vi "RDV-addDataToMap.vi"(7 "Use ignore list (false)":bool, 8 "error in (no error)":errorcluster, 9 "data":T2[](array[typedef]), 10 "all data":cluster{"key":string, "data":T1}[](array[cluster]), 11 "RDV-Reflection_Data_viewer in":refnum<class "RDV-Reflection_Data_viewer.lvclass">) -> (0 "error out":errorcluster, 3 "RDV-Reflection_Data_viewer out":refnum<class "RDV-Reflection_Data_viewer.lvclass">)   [LabVIEW 2020, in "RDV-Reflection_Data_viewer.lvclass"]
doc: "Adds data clusters with their keys to the viewer's data map. Use ignore list skips keys on the ignore list."
uses:
  RDV-Reflection_Data_viewer.lvclass
  Reflector/RFH-common_data_format.ctl
  RDV-DATA_MAP_CLUST.ctl
  RDV-Reflection_Data_viewer.lvclass/RDV-Reflection_Data_viewer.ctl
  Reflector/RFH-Reflection_File_Handler.lvlib
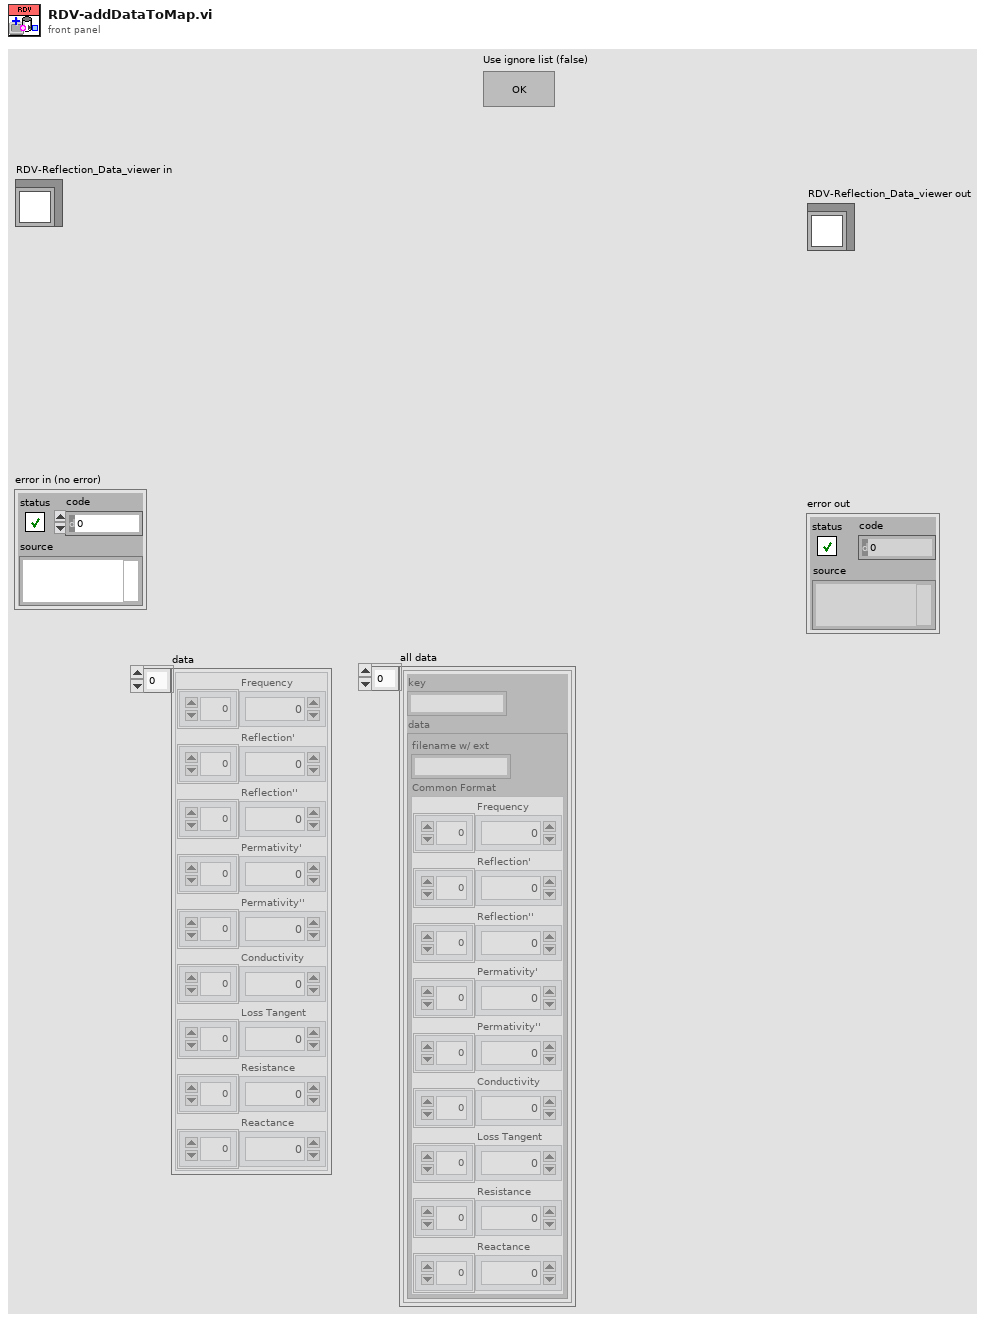
[diagram p1: front panel]
types:
  T1 = typedef "RDV-Reflection_Data_viewer.lvclass/RDV-DATA_MAP_CLUST.ctl" = cluster{"filename w/ ext":string, "Common Format":T2}
  T2 = typedef "RFH-Reflection_File_Handler.lvlib/RFH-common_data_format.ctl" = cluster{"Frequency":dbl[], "Reflection'":dbl[], "Reflection''":dbl[], "Permativity'":dbl[], "Permativity''":dbl[], "Conductivity":dbl[], "Loss Tangent":dbl[], "Resistance":dbl[], "Reactance":dbl[]}
  T3 = typedef "RDV-Reflection_Data_viewer.lvclass/RDV-UPDATE_IGNORE_LIST.ctl" = string[]
  T4 = typedef "RDV-Reflection_Data_viewer.lvclass/RDV-DATA_MAP.ctl" = map{string, T1}
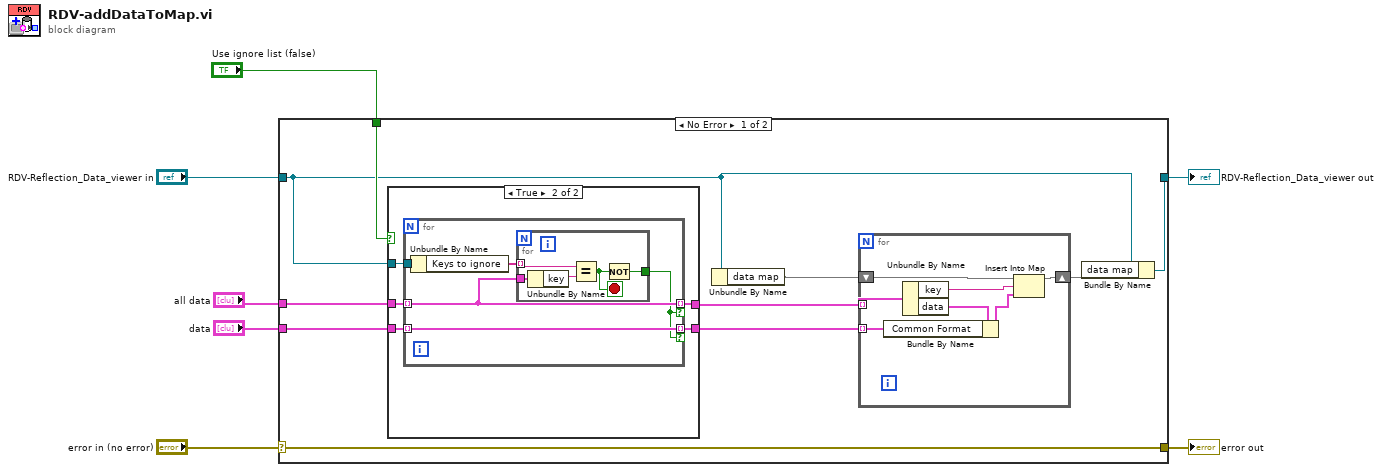
[diagram p0: block diagram]
diagram:
  n1 = case shown="No Error" "error in (no error)" {
    selector: "error in (no error)" -> [w14 w43]
    tunnel: [w14 w43] -> w6
    tunnel: [w15 w42] -> w4
    tunnel: "RDV-Reflection_Data_viewer in" -> [w8 w42]
    tunnel: "all data" -> [w12 _]
    tunnel: "data" -> [w13 _]
    tunnel: "Use ignore list (false)" -> [w9 _]
    frame No Error {
      n2 = case shown="True" w9 {
        tunnel: w13 -> [w18 w24]
        tunnel: w12 -> [w19 w23]
        tunnel: [w19 w22] -> w11
        tunnel: [w18 w21] -> w10
        tunnel: w8 -> [_ w20]
        frame False {
        }
        frame True {
          n3 = for {
            tunnel: w24 -> [w29] mode=indexing
            tunnel: w23 -> [w26] mode=indexing
            tunnel: [w26] -> w22 mode=indexing if=w25
            tunnel: [w29] -> w21 mode=indexing if=w25
            tunnel: w20 -> [w28]
            n4 = Unbundle By Name(w28) -> ("Keys to ignore"=w27:T3)
            n5 = for {
              tunnel: w27 -> [w32] mode=indexing
              tunnel: w26 -> [w34]
              tunnel: [w31] -> w25
              stop <- w30 stop-if-true
              n6 = Unbundle By Name(w34) -> ("key"=w33:string)
              n7 = Equal?(x=w32, y=w33) -> (x = y?=w30:bool)
              n8 = Not(x=w30) -> (.not. x?=w31:bool)
            }
          }
        }
      }
      n9 = Unbundle By Name(w8) -> ("data map"=w17:T4)
      n10 = for {
        shift-right: [w40] -> w16
        shift-left: w17 -> [w41]
        tunnel: w11 -> [w39] mode=indexing
        tunnel: w10 -> [w35] mode=indexing
        n11 = Unbundle By Name(w39) -> ("key"=w37:string, "data"=w38:T1)
        n12 = Bundle By Name(cluster=w38, "Common Format"=w35) -> (w36:T1)
        n13 = Insert Into Map(map in=w41, key=w37, value=w36) -> (map out=w40:T4)  [unwired: 2 out]
      }
      n14 = Bundle By Name(cluster=w8, "data map"=w16) -> (w15:refnum<class "RDV-Reflection_Data_viewer.lvclass">)
    }
    frame Error {
    }
  }
  "error out" <- w6
  "RDV-Reflection_Data_viewer out" <- w4
